vi "RGBToHSV.vi"(1 "RBG U32":u32) -> (0 "HSV":u16)   [LabVIEW 2024]
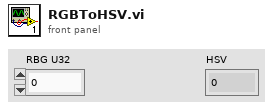
[diagram p1: front panel]
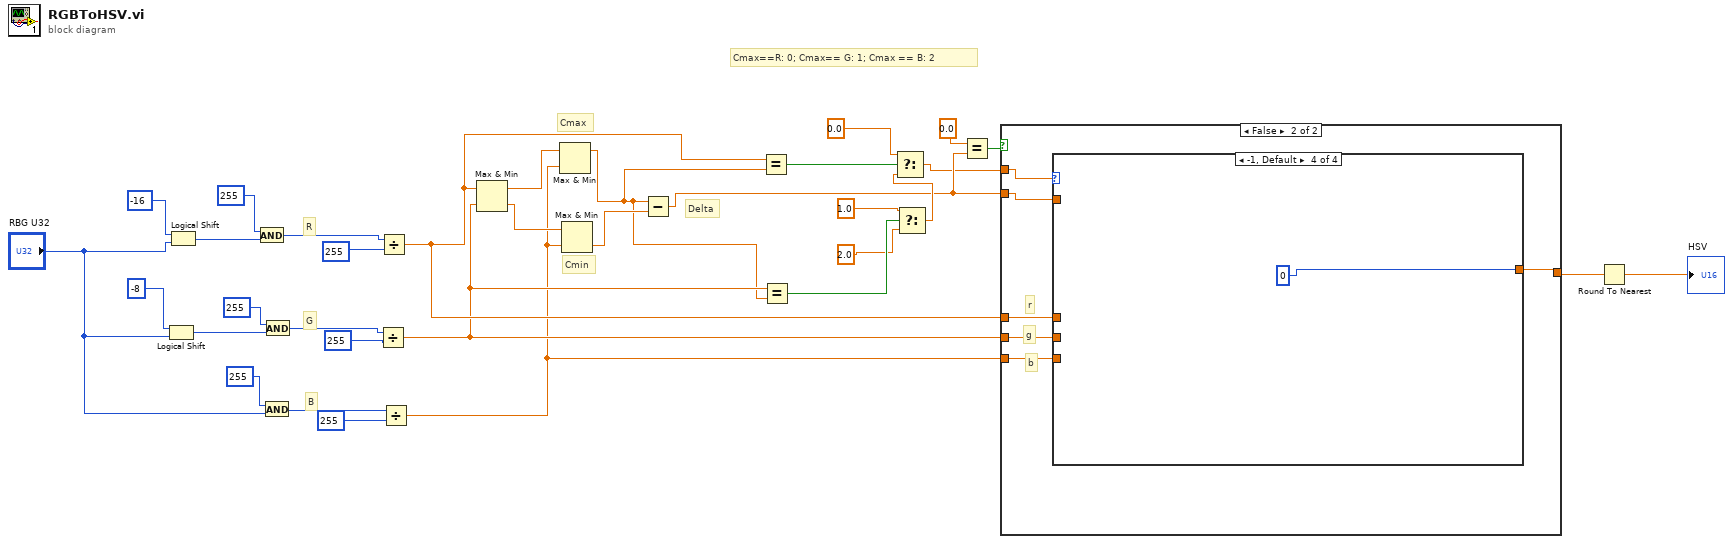
[diagram p0: block diagram]
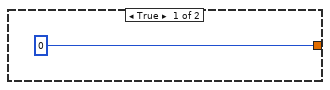
[diagram p2: hidden frame]
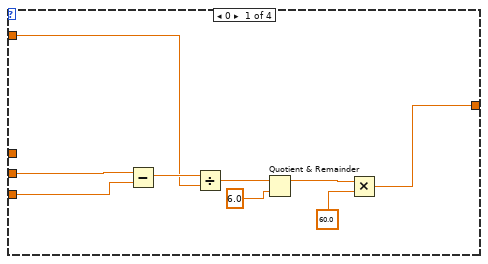
[diagram p3: hidden frame]
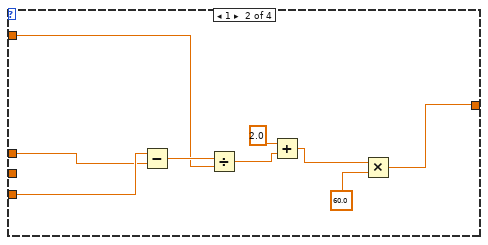
[diagram p4: hidden frame]
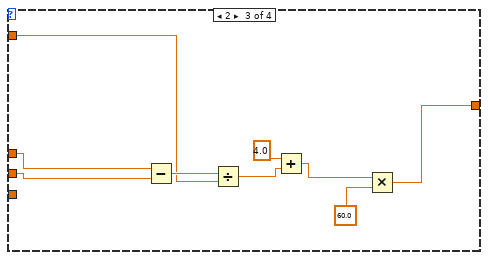
[diagram p5: hidden frame]
diagram:
  # "Delta"
  # "Cmax==R: 0; Cmax== G: 1; Cmax == B: 2"
  # "Cmin"
  # "Cmax"
  # "B"
  # "G"
  # "R"
  n1 = Logical Shift(y=i16 -8, x="RBG U32") -> (x << y=w29:u32)
  n2 = Logical Shift(y=i8 -16 ("x"), x="RBG U32") -> (x << y=w31:u32)
  n3 = And(x=u32 255, y=w31) -> (x .and. y?=w25:u32)
  n4 = And(x=u32 255, y="RBG U32") -> (x .and. y?=w23:u32)
  n5 = And(x=u32 255, y=w29) -> (x .and. y?=w24:u32)
  n6 = Divide(x=w24, y=u32 255) -> (x/y=w9:dbl)
  n7 = Divide(x=w25, y=u32 255) -> (x/y=w10:dbl)
  n8 = Divide(x=w23, y=u32 255) -> (x/y=w8:dbl)
  n9 = Max & Min(x=w10, y=w9) -> (max(x,y)=w18:dbl, min(x,y)=w19:dbl)
  n10 = Max & Min(x=w18, y=w8) -> (max(x,y)=w7:dbl)  [unwired: 1 out]
  n11 = Max & Min(x=w19, y=w8) -> (min(x,y)=w17:dbl)  [unwired: 1 out]
  n12 = Subtract(x=w7, y=w17) -> (x-y=w5:dbl)
  n13 = Equal?(x=w10, y=w7) -> (x = y?=w16:bool)
  n14 = Equal?(x=w9, y=w7) -> (x = y?=w13:bool)
  n15 = Select(t=1.0, s=w13, f=2.0) -> (s? t:f=w14:dbl)
  n16 = Select(t=0.0, s=w16, f=w14) -> (s? t:f=w3:dbl)
  n17 = Equal?(x=0.0, y=w5) -> (x = y?=w6:bool)
  n18 = case shown="False" w6 {
    tunnel: w10 -> [_ w38]
    tunnel: w9 -> [_ w37]
    tunnel: w8 -> [_ w36]
    tunnel: w5 -> [_ w39]
    tunnel: w3 -> [_ w40]
    tunnel: [0 w35] -> w2
    frame True {
    }
    frame False {
      # "b"
      # "g"
      # "r"
      n19 = case shown="-1, Default" w40 {
        tunnel: w39 -> [w46 w54 w59 _]
        tunnel: w38 -> [_ w56 w61 _]
        tunnel: w37 -> [w49 _ w60 _]
        tunnel: w36 -> [w48 w57 _ _]
        tunnel: [w41 w50 w62 0] -> w35
        frame 0 {
          n20 = Subtract(x=w49, y=w48) -> (x-y=w47:dbl)
          n21 = Divide(x=w47, y=w46) -> (x/y=w45:dbl)
          n22 = Quotient & Remainder(x=w45, y=6.0) -> (x-y*floor(x/y)=w43:dbl)  [unwired: 1 out]
          n23 = Multiply(x=w43, y=60.0) -> (x*y=w41:dbl)
        }
        frame 1 {
          n24 = Subtract(x=w57, y=w56) -> (x-y=w55:dbl)
          n25 = Divide(x=w55, y=w54) -> (x/y=w52:dbl)
          n26 = Add(x=2.0, y=w52) -> (x+y=w51:dbl)
          n27 = Multiply(x=w51, y=60.0) -> (x*y=w50:dbl)
        }
        frame 2 {
          n28 = Subtract(x=w61, y=w60) -> (x-y=w66:dbl)
          n29 = Divide(x=w66, y=w59) -> (x/y=w64:dbl)
          n30 = Add(x=4.0, y=w64) -> (x+y=w63:dbl)
          n31 = Multiply(x=w63, y=60.0) -> (x*y=w62:dbl)
        }
        frame -1, Default {
        }
      }
    }
  }
  n32 = Round To Nearest(number=w2) -> (nearest integer value=→"HSV":dbl)
